vi "Open Project.vi"(7 "Open Project Window ?":bool, 8 "error in (no error)":errorcluster, 10 "Project Path in":path) -> (0 "error out":errorcluster, 3 "Project out":refnum<vi>)   [LabVIEW 2019, in "gRPC Template Creation Utility.lvlib"]
uses:
  gRPC Template Creation Utility.lvlib
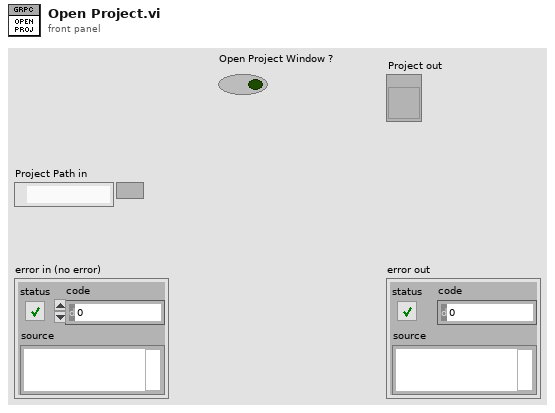
[diagram p1: front panel]
types:
  T1 = enum32{"invalid app kind", "Development System", "Run Time System", "Student Edition", "Embedded LabVIEW", "Evaluation", "Custom"}
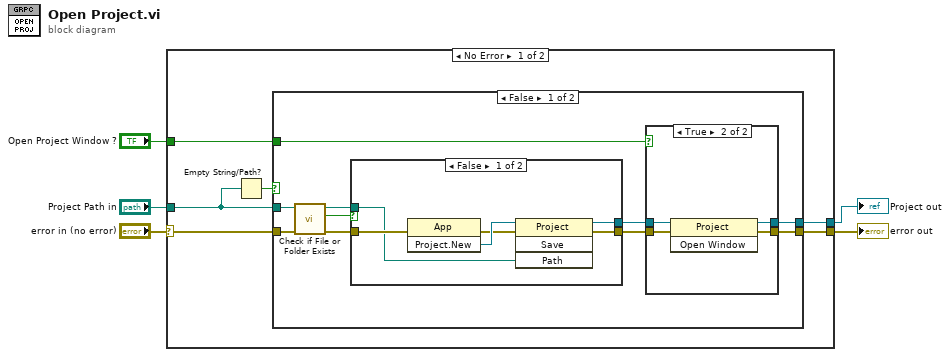
[diagram p0: block diagram]
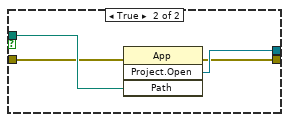
[diagram p3: hidden frame]
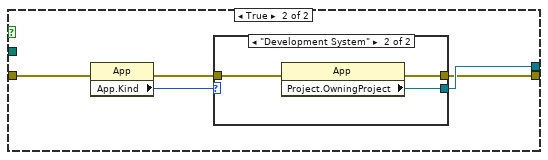
[diagram p4: hidden frame]
diagram:
  n1 = case shown="No Error" "error in (no error)" {
    selector: "error in (no error)" -> [w9 w47]
    tunnel: "Project Path in" -> [w7 _]
    tunnel: "Open Project Window ?" -> [w8 _]
    tunnel: [w11 _] -> w3
    tunnel: [w10 w47] -> w2
    frame No Error {
      n2 = Empty String/Path?(string/path=w7) -> (empty?=w6:bool)
      n3 = case shown="False" w6 {
        tunnel: w7 -> [w21 _]
        tunnel: [w15 w42] -> w11
        tunnel: [w14 w41] -> w10
        tunnel: w9 -> [w13 w39]
        tunnel: w8 -> [w12 _]
        frame False {
          n4 = call <vilib>:"Check if File or Folder Exists.vi"("error in (no error)"=w13, "path"=w21) -> ("error out"=w18:errorcluster, "file or folder exists?"=w19:bool, "dup path"=w20:path)  [unwired: 7 in]
          n5 = case shown="False" w19 {
            tunnel: [w29 w35] -> w17
            tunnel: w20 -> [w30 w37]
            tunnel: w18 -> [w32 w36]
            tunnel: [w28 w34] -> w16
            frame False {
              n6 = invoke class="App" method="Project.New"(error in=w32) -> (error out=w31:errorcluster, "Project:New"=w33:refnum<vi>)  [unwired: 2 in, 1 out]
              n7 = invoke class="Project" method="Save"(reference=w33, error in=w31, "Path"=w30) -> (reference out=w29:refnum<vi>, error out=w28:errorcluster)  [unwired: 1 in, 2 out]
            }
            frame True {
              n8 = invoke class="App" method="Project.Open"(error in=w36, "Path"=w37) -> (error out=w34:errorcluster, "Project:Open"=w35:refnum<vi>)  [unwired: 2 in, 2 out]
            }
          }
          n9 = case shown="True" w12 {
            tunnel: w17 -> [w23 w27]
            tunnel: w16 -> [w22 w26]
            tunnel: [w23 w25] -> w15
            tunnel: [w22 w24] -> w14
            frame False {
            }
            frame True {
              n10 = invoke class="Project" method="Open Window"(reference=w27, error in=w26) -> (reference out=w25:refnum<vi>, error out=w24:errorcluster)  [unwired: 1 in, 1 out]
            }
          }
        }
        frame True {
          n11 = property class="App"(error in=w39) -> (error out=w38:errorcluster, "App.Kind"=w40:T1)  [unwired: 1 in, 1 out]
          n12 = case shown="\"Development System\"" w40 {
            tunnel: [_ w46] -> w42
            tunnel: [w43 w45] -> w41
            tunnel: w38 -> [w43 w44]
            frame "invalid app kind", Default {
            }
            frame "Development System" {
              n13 = property class="App"(error in=w44) -> (error out=w45:errorcluster, "Project.OwningProject"=w46:refnum<vi>)  [unwired: 1 in, 1 out]
            }
          }
        }
      }
    }
    frame Error {
    }
  }
  "Project out" <- w3
  "error out" <- w2
